vi "VM - Destroy Variable.vi"(7 "VC Handle":T2=-1, 8 "error in":errorcluster, 9 "global ? (F)":bool, 11 "name_spec":string) -> (0 "error out":errorcluster, 1 "err code":T1 items=["No error", "Invalid variable type", "Variable not found", "Variable already exists", "Invalid context handle", "Input error", "Invalid data format", "No history attached", "History already attached", "Invalid history parameters", "Wrong variable name", "Wrong alias name", "Non-unique alias", "Alias not found", "No alias associated", "Alias already associated", "Wrong context name", "Non-unique context name", "Context name not found", "Invalid parameter", "Generic error", "Memory Full", "Unrecognized LV error", "Unknown error code"], 3 "dup name_spec":string, 5 "dup VC Handle":T2=-1)   [LabVIEW 2021]
doc: "This VI destroys a variable of any data type. Refer to the VI help for more details.\n\n<b>VC Handle</b> specifies the handle of the variable context. This input is ignored if the <b>name_spec</b> control refers to a variable by an alias or if the <b>global?</b> control is TRUE.\n\n<b>name_spec</b> is the name specifier of the desired variable. Usually, it is merely a variable name; however, its generic format is '[name][=alias]', where either 'name' or '=alias' can be omitted but not both.\n\n<b>global?</b> control, if TRUE, causes the VI to ignore <b>VC Handle</b> and operate on a global variable.\n\n<b>err code</b> indicator returns a VarMan Engine error code.\n\n::: CalcExpress Toolkit :::\nCopyright (c) 2000-2026 Konstantin Shifershteyn. All rights reserved."
uses:
  cetypes.llb/VarMan Variable Context Handle.ctl
  cetypes.llb/VarMan Error Code.ctl
  cersrc/celveng32.dll
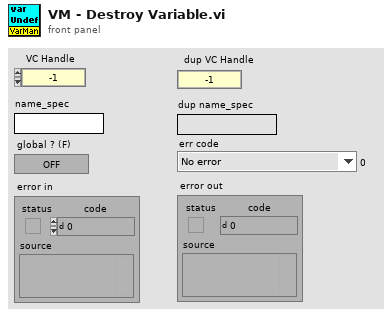
[diagram p1: front panel]
types:
  T1 = typedef "VarMan Error Code.ctl" = u16
  T2 = typedef "VarMan Variable Context Handle.ctl" = i32
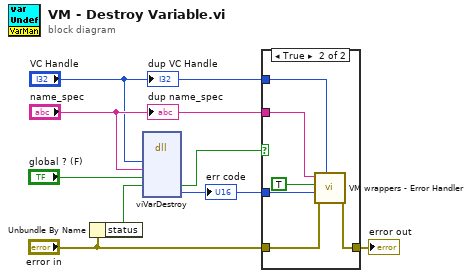
[diagram p0: block diagram]
diagram:
  n1 = Unbundle By Name("error in") -> ("status"=w5:bool)
  n2 = dll-call lib="C:/LV Projects/CalcExpress 40 LV2021/vi.lib/addons/CalcExpress/cersrc/celveng*.dll" fn="viVarDestroy"("vch"="VC Handle", "name"="name_spec", "gbl"="global ? (F)", "errf"=w5) -> ("errf"=w1:bool, "err code"=w4:T1)  [unwired: 8 in, 2 out]
  "err code" <- w4
  n3 = case shown="True" w1 {
    tunnel: [w9 w15] -> w8
    tunnel: "error in" -> [w9 w14]
    tunnel: w4 -> [_ w12]
    tunnel: "name_spec" -> [_ w13]
    tunnel: "VC Handle" -> [_ w10]
    frame False {
    }
    frame True {
      n4 = call "VM wrappers - Error Handler.vi"("VC Handle"=w10, "error before"=w14, "VarMan error"=w12, "show name spec (F)"=TRUE, "name spec"=w13) -> ("error out"=w15:errorcluster)  [unwired: 5 in, 1 out]
    }
  }
  "error out" <- w8
  "dup VC Handle" <- "VC Handle"
  "dup name_spec" <- "name_spec"
